vi "Func - Prepare argument descriptors.vi"(5 "number":i32, 6 "error in":bool, 8 "arg templates":T1(array[cluster]), 9 "arg descriptors in":T1(array[cluster])) -> (0 "error out":bool, 3 "arg descriptors out":T1(array[cluster]))   [LabVIEW 2021]
doc: "::: CalcExpress Toolkit :::\nCopyright (c) 2000-2026 Konstantin Shifershteyn. All rights reserved."
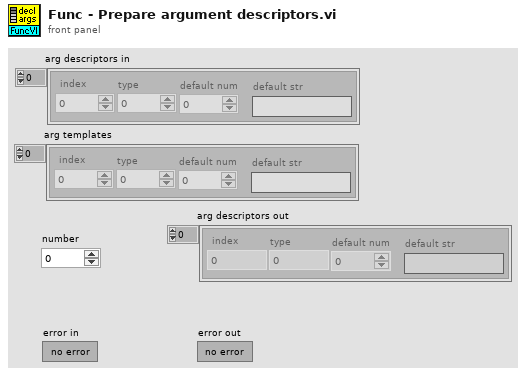
[diagram p1: front panel]
types:
  T1 = cluster{"index":i32, "type":i32, "default num":dbl, "default str":string}[]
  T2 = cluster{"index":i32, "type":i32, "default num":dbl, "default str":string}
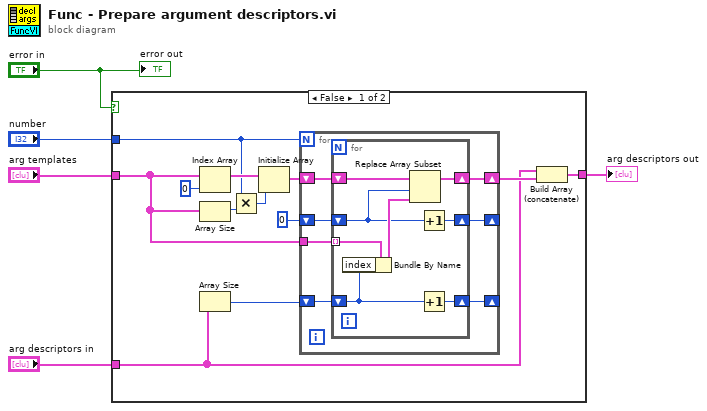
[diagram p0: block diagram]
diagram:
  n1 = case shown="False" "error in" {
    tunnel: [w10 w33] -> w5
    tunnel: "arg descriptors in" -> [w8 w33]
    tunnel: "arg templates" -> [w7 _]
    tunnel: "number" -> [w6 _]
    frame False {
      n2 = Index Array(array=w7, index=0) -> (element=w14:T2)
      n3 = Array Size(array=w7) -> (size(s)=w16:i32)
      n4 = Array Size(array=w8) -> (size(s)=w9:i32)
      n5 = Multiply(x=w6, y=w16) -> (x*y=w15:i32)
      n6 = Initialize Array(w14, w15) -> (w17:T1)
      n7 = for {
        N: w6 -> [_]
        tunnel: w7 -> [w24]
        shift-right: [w22] -> _
        shift-left: w9 -> [w23]
        shift-right: [w18] -> w11
        shift-left: w17 -> [w21]
        shift-right: [w19] -> _
        shift-left: 0 -> [w20]
        n8 = for {
          tunnel: w24 -> [w32] mode=indexing
          shift-right: [w31] -> w22
          shift-left: w23 -> [w30]
          shift-right: [w26] -> w18
          shift-left: w21 -> [w29]
          shift-right: [w27] -> w19
          shift-left: w20 -> [w25]
          n9 = Bundle By Name(cluster=w32, "index"=w30) -> (w28:T2)
          n10 = Replace Array Subset(array=w29, new element=w28, index=w25) -> (w26:T1)
          n11 = Increment(x=w25) -> (x+1=w27:i32)
          n12 = Increment(x=w30) -> (x+1=w31:i32)
        }
      }
      n13 = Build Array (concatenate)(w8, w11) -> (w10:T1)
    }
    frame True {
    }
  }
  "arg descriptors out" <- w5
  "error out" <- "error in"
